vi "Write_Echo.vi"(7 "new id":u32 format="%.0x", 8 "error in (no error)":errorcluster, 9 "i":i32, 10 "frames":T1 {"flags" format="%.0x"; "id" format="%.0x"}, 11 "channel in":refnum<class "CANsub_DirectChannel.lvclass">) -> (0 "error out":errorcluster, 3 "channel out":refnum<class "CANsub_DirectChannel.lvclass">)   [LabVIEW 2021, in "CANsub_API.lvlib" / "CANsub_DirectChannel.lvclass"]
doc: "Direct: Check_Open ? W14 C_Echo_RT (frame i of frames, new ID, keeps IDE/FDF/BRS) into the TX buffer (in place) ? Send_TX. Loop-safe: no allocation, bounded time."
uses:
  CANsub_DirectChannel.lvclass
  CANsub_DirectChannel.lvclass/CANsub_DirectChannel.ctl
  CANsub_API.lvlib
  CANsub_C.lvlib
  Typedefs/CANsub_Frames.ctl
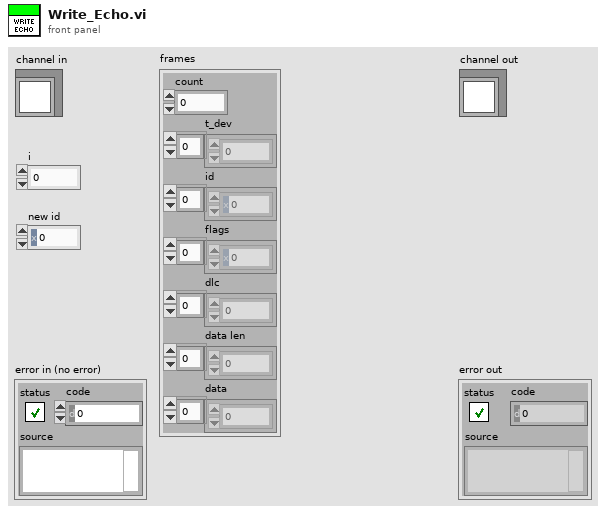
[diagram p1: front panel]
types:
  T1 = typedef "CANsub_API.lvlib/CANsub_Frames.ctl" = cluster{"count":i32, "t_dev":dbl[], "id":u32[], "flags":u16[], "dlc":u8[], "data len":u8[], "data":u8[]}
  T2 = typedef "CANsub_API.lvlib/CANsub_Status.ctl" = cluster{"state":T3, "frames read":u32, "frames written":u32, "crc errors":u32, "decode errors":i32, "pings":u32, "FIFO overflows":u32, "reopens":u32, "nodelay":i32, "api version":string, "lib version":u32, "bit timing":T4, "last error":errorcluster}
  T3 = typedef "CANsub_API.lvlib/CANsub_State.ctl" = enum16{"Closed", "Open", "Lost"}
  T4 = typedef "CANsub_Common.lvlib/Bit_Timing.ctl" = cluster{"brp":u16, "seg1":u16, "seg2":u16, "sjw":u16, "data brp":u16, "data seg1":u16, "data seg2":u16, "data sjw":u16}
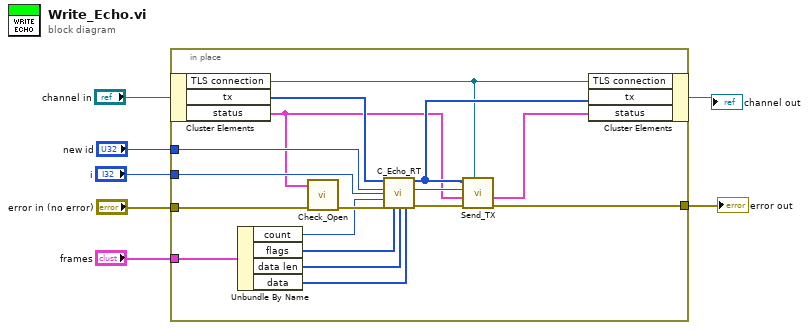
[diagram p0: block diagram]
diagram:
  n1 = in-place {
    in-place-border: "error in (no error)" -> [w24]
    in-place-border: "frames" -> [w23]
    in-place-border: "i" -> [w20]
    in-place-border: "new id" -> [w19]
    in-place-border: [w8] -> w1
    n2 = in-place-cluster #1("channel in") -> ("TLS connection"=w10:refnum<k5>, "tx"=w21:u8[], "status"=w11:T2)
    n3 = Unbundle By Name(w23) -> ("count"=w18:i32, "flags"=w17:u16[], "data len"=w16:u8[], "data"=w15:u8[])
    n4 = call "Check_Open.vi"("error in (no error)"=w24, "status"=w11) -> ("error out"=w22:errorcluster)  [unwired: 9 in]
    n5 = call "C_Echo_RT.vi"("tx in"=w21, "flags"=w17, "data len"=w16, "data"=w15, "new id"=w19, "index"=w20, "n frames"=w18, "error in (no error)"=w22) -> ("tx out"=w13:u8[], "length"=w12:i32, "error out"=w14:errorcluster)  [unwired: 5 in]
    n6 = call "Send_TX.vi"("TLS connection"=w10, "error in (no error)"=w14, "status in"=w11, "length"=w12, "tx"=w13) -> ("error out"=w8:errorcluster, "status out"=w9:T2)  [unwired: 5 in]
    n7 = in-place-cluster #1("TLS connection"=w10, "tx"=w13, "status"=w9) -> (→"channel out":refnum<class "CANsub_DirectChannel.lvclass">)
  }
  "error out" <- w1
